vi "State_Machine_Latched.vi"(0 "Current State":T1, 1 "Tilt":bool, 2 "Motion":bool, 3 "State Elapsed (s)":dbl, 4 "Cancel":bool, 5 "Reset":bool, 7 "error in (no error)":errorcluster caption="错误输入（无错误）", 8 "Suspect Delay (s)":dbl=5.0 format="%#_13g", 10 "Countdown Duration (s)":dbl=30.0 format="%#_13g") -> (20 "Next State":T1, 21 "Countdown":dbl, 22 "Alarm":bool, 27 "error out":errorcluster caption="错误输出")   [LabVIEW 2020]
doc: "PLACEHOLDER: error interface only. Fall detection state logic NOT implemented."
uses:
  Controls/State.ctl
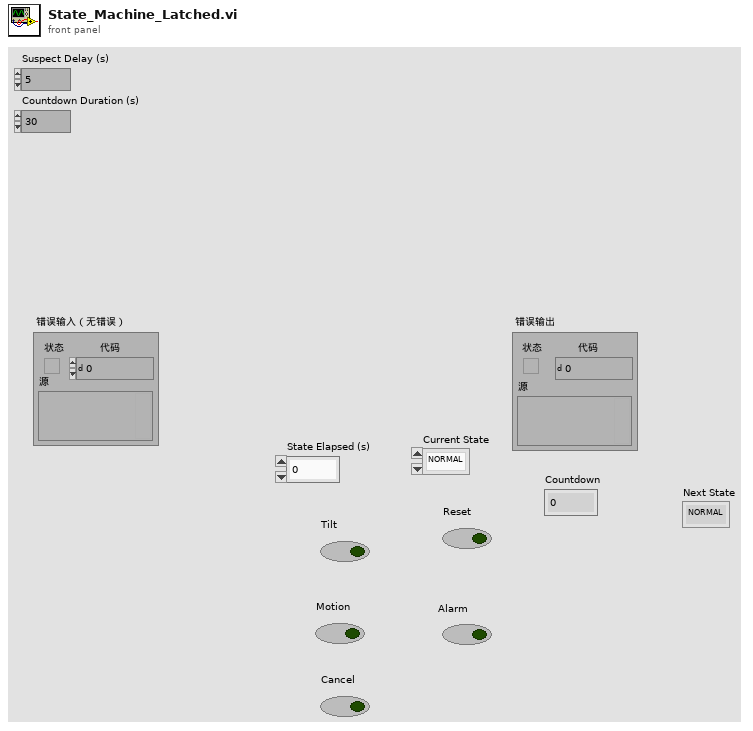
[diagram p1: front panel]
types:
  T1 = typedef "State.ctl" = enum16{"NORMAL", "SUSPECT", "COUNTDOWN", "ALARM", "RESET"}
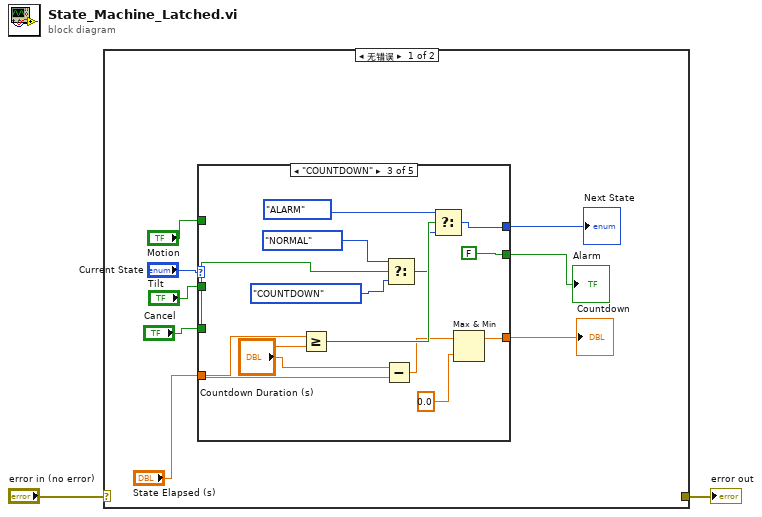
[diagram p0: block diagram]
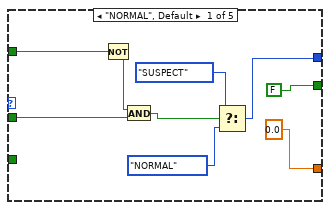
[diagram p2: hidden frame]
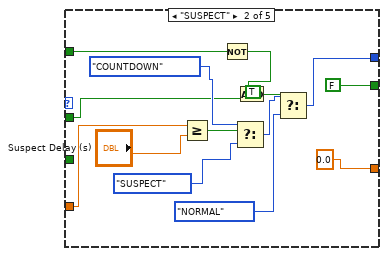
[diagram p3: hidden frame]
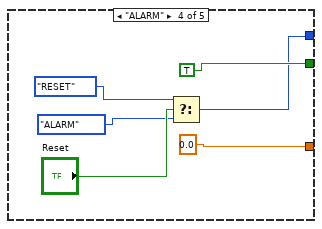
[diagram p4: hidden frame]
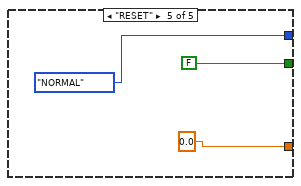
[diagram p5: hidden frame]
diagram:
  n1 = case shown="无错误" "error in (no error)" {
    selector: "error in (no error)" -> [_ w56]
    tunnel: [_ w56] -> w1
    frame No Error {
      n2 = case shown="\"COUNTDOWN\"" "Current State" {
        tunnel: [FALSE ("Alarm") FALSE FALSE TRUE FALSE] -> w9
        tunnel: [0.0 ("Countdown") 0.0 w38 0.0 0.0] -> w8
        tunnel: [w15 w30 w39 w47 State."NORMAL" ("枚举")] -> w7
        tunnel: "Motion" -> [w12 w26 _ _ _]
        tunnel: "Tilt" -> [w11 w25 _ _ _]
        tunnel: "State Elapsed (s)" -> [_ w22 w35 _ _]
        tunnel: "Cancel" -> [_ _ w45 _ _]
        frame "NORMAL", Default {
          n3 = Not(x=w12) -> (.not. x?=w13:bool)
          n4 = And(x=w13, y=w11) -> (x .and. y?=w14:bool)
          n5 = Select(t=State."SUSPECT" ("枚举"), s=w14, f=State."NORMAL" ("枚举")) -> (s? t:f=w15:T1)
        }
        frame "SUSPECT" {
          (unwired) TRUE
          n6 = Greater Or Equal?(x=w22, y="Suspect Delay (s)") -> (x >= y?=w21:bool)
          n7 = Not(x=w26) -> (.not. x?=w27:bool)
          n8 = Select(t=State."COUNTDOWN" ("枚举"), s=w21, f=State."SUSPECT" ("枚举")) -> (s? t:f=w23:T1)
          n9 = And(x=w27, y=w25) -> (x .and. y?=w20:bool)
          n10 = Select(t=w23, s=w20, f=State."NORMAL" ("枚举")) -> (s? t:f=w30:T1)
        }
        frame "COUNTDOWN" {
          n11 = Greater Or Equal?(x=w35, y="Countdown Duration (s)") -> (x >= y?=w42:bool)
          n12 = Subtract(x="Countdown Duration (s)", y=w35) -> (x-y=w36:dbl)
          n13 = Select(t=State."NORMAL" ("枚举"), s=w45, f=State."COUNTDOWN" ("枚举")) -> (s? t:f=w40:T1)
          n14 = Select(t=State."ALARM" ("枚举"), s=w42, f=w40) -> (s? t:f=w39:T1)
          n15 = Max & Min(x=w36, y=0.0) -> (max(x,y)=w38:dbl)  [unwired: 1 out]
        }
        frame "ALARM" {
          n16 = Select(t=State."RESET" ("枚举"), s="Reset", f=State."ALARM" ("枚举")) -> (s? t:f=w47:T1)
        }
        frame "RESET" {
        }
      }
      "Next State" <- w7
      "Alarm" <- w9
      "Countdown" <- w8
    }
    frame Error {
    }
  }
  "error out" <- w1
